vi "Mark InBand.vi"(8 "error in (no error)":errorcluster caption="에러 입력(에러 없음)", 10 "Limit":dbl, 11 "Instrument Manager 입력":refnum<class "Instrument Manager.lvclass">) -> (0 "error out":errorcluster caption="에러 출력", 2 "amplitude":dbl, 3 "Instrument Manager 출력":refnum<class "Instrument Manager.lvclass">)   [LabVIEW 2023, in "Instrument Manager.lvclass"]
uses:
  Instrument Manager.lvclass
  Instrument Manager.lvclass/Instrument Manager.ctl
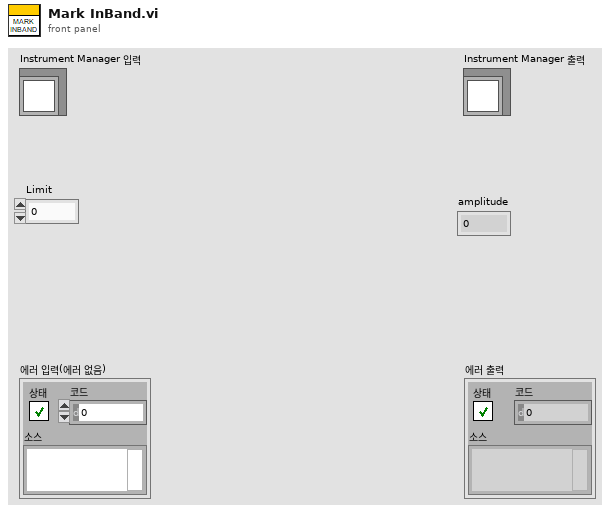
[diagram p1: front panel]
types:
  T1 = typedef "Spectrum Analyzer.lvlib/TYPE Marker Value.ctl" = cluster{"X-axis":dbl, "Y-axis":dbl}
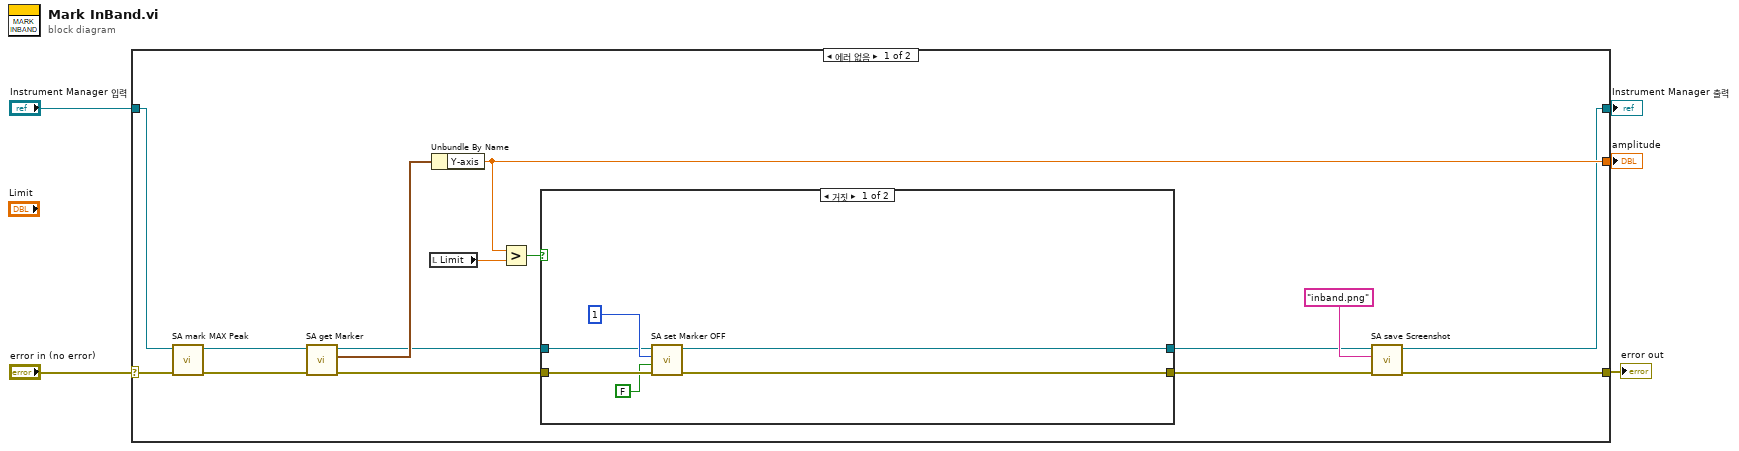
[diagram p0: block diagram]
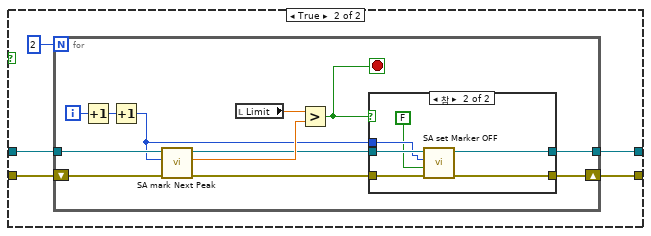
[diagram p2: hidden frame]
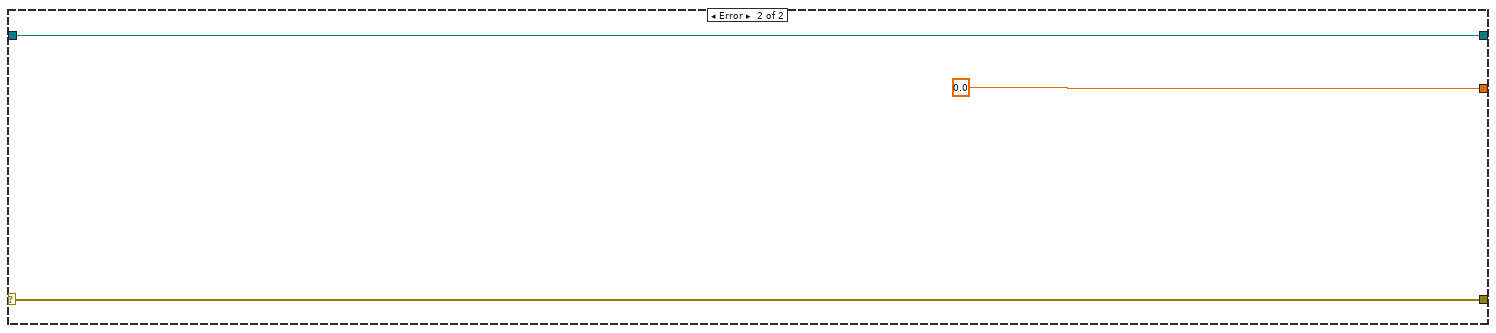
[diagram p4: hidden frame]
diagram:
  n1 = case shown="에러 없음" "error in (no error)" {
    selector: "error in (no error)" -> [w19 w54]
    tunnel: [w8 w54] -> w4
    tunnel: [w6 w53] -> w2
    tunnel: "Instrument Manager 입력" -> [w18 w53]
    tunnel: [w11 0.0 ("Y-axis")] -> w1
    frame No Error {
      n2 = call "SA mark MAX Peak.vi"("error in (no error)"=w19, "Instrument Manager 입력"=w18) -> ("error out"=w20:errorcluster, "Instrument Manager 출력"=w17:refnum<class "Instrument Manager.lvclass">)  [unwired: 8 in]
      n3 = call "SA get Marker.vi"("error in (no error)"=w20, "Instrument Manager 입력"=w17) -> ("error out"=w16:errorcluster, "Marker Value"=w15:T1, "Instrument Manager 출력"=w12:refnum<class "Instrument Manager.lvclass">)  [unwired: 7 in]
      n4 = local read "Limit"() -> (w14:dbl)
      n5 = Unbundle By Name(w15) -> ("Y-axis"=w11:dbl)
      n6 = Greater?(x=w11, y=w14) -> (0:w13:bool)
      n7 = case shown="거짓" w13 {
        tunnel: w16 -> [w24 w31]
        tunnel: w12 -> [w25 w30]
        tunnel: [w22 w28] -> w7
        tunnel: [w23 w27] -> w9
        frame False {
          n8 = call "SA set Marker OFF.vi"("error in (no error)"=w24, "On?"=FALSE, "Marker Index"=1, "Instrument Manager 입력"=w25) -> ("error out"=w23:errorcluster, "Instrument Manager 출력"=w22:refnum<class "Instrument Manager.lvclass">)  [unwired: 6 in]
        }
        frame True {
          n9 = for {
            N: 2 -> [_]
            tunnel: w30 -> [w42]
            shift-right: [w35] -> w27
            shift-left: w31 -> [w43]
            tunnel: [w34] -> w28
            i -> [w41]
            stop <- w33 stop-if-true
            n10 = Increment(x=w41) -> (x+1=w40:i32)
            n11 = Increment(x=w40) -> (x+1=w32:i32)
            n12 = call "SA mark Next Peak.vi"("error in (no error)"=w43, "Marker Index"=w32, "Instrument Manager 입력"=w42) -> ("error out"=w37:errorcluster, "Amplitude"=w38:dbl, "Instrument Manager 출력"=w36:refnum<class "Instrument Manager.lvclass">)  [unwired: 6 in]
            n13 = local read "Limit"() -> (w39:dbl)
            n14 = Greater?(x=w39, y=w38) -> (0:w33:bool)
            n15 = case shown="참" w33 {
              tunnel: w37 -> [w44 w51]
              tunnel: w36 -> [w45 w50]
              tunnel: [w44 w49] -> w35
              tunnel: [w45 w48] -> w34
              tunnel: w32 -> [_ w47]
              frame False {
              }
              frame True {
                n16 = call "SA set Marker OFF.vi"("error in (no error)"=w51, "On?"=FALSE, "Marker Index"=w47, "Instrument Manager 입력"=w50) -> ("error out"=w49:errorcluster, "Instrument Manager 출력"=w48:refnum<class "Instrument Manager.lvclass">)  [unwired: 6 in]
              }
            }
          }
        }
      }
      n17 = call "SA save Screenshot.vi"("error in (no error)"=w9, "File Name"="inband.png", "Instrument Manager 입력"=w7) -> ("error out"=w8:errorcluster, "Instrument Manager 출력"=w6:refnum<class "Instrument Manager.lvclass">)  [unwired: 7 in]
    }
    frame Error {
    }
  }
  "error out" <- w4
  "Instrument Manager 출력" <- w2
  "amplitude" <- w1
